vi "ChangeInheritanceDialog.vi"(0 "ClassWriterGOOP300 in":refnum<class "ClassWriterNative.lvclass">, 1 "LvClass":refnum<vi>, 5 "error in (no error)":errorcluster) -> (14 "ClassWriterGOOP300 out":refnum<class "ClassWriterNative.lvclass">, 15 "BaseClassPath":path, 16 "Cancelled":bool, 19 "error out":errorcluster)   [LabVIEW 2020, in "ClassWriterNative.lvclass"]
uses:
  ClassWriterNative.lvclass
  SubVIs/GOOP_HelpButton.ctl
panel:
  in  "Change inheritance to this class":string(combo)
  in  "_HelpChangeInheritance":T1
  in  "_Cancel":bool
  in  "_OK":bool
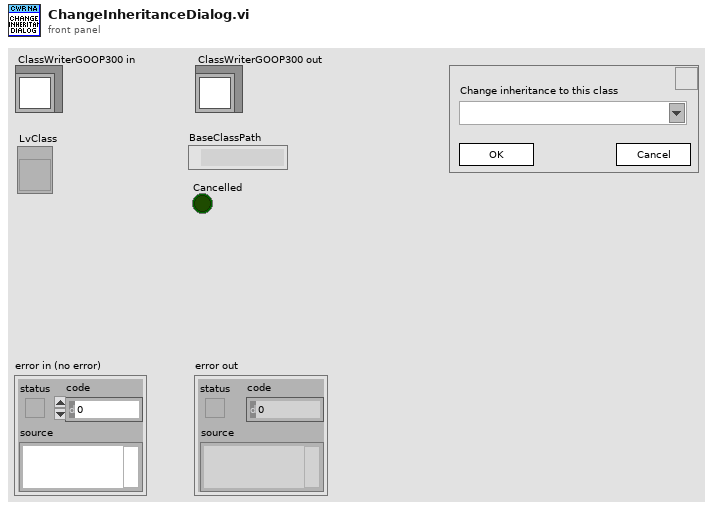
[diagram p1: front panel]
types:
  T1 = typedef "GOOP_HelpButton.ctl" = bool
  T2 = cluster{"LvClasses":refnum<vi>[], "ClassPathes":path[], "Cancelled":bool, "List":string[], "List index":i32}
  T3 = typedef "GDSLvCLass_ClassSettingsType.ctl" = cluster{"ClassProviderName":string, "ClassTemplateUsed":string, "ClassTemplateVersion":string, "ClassDescription":string, "PlugIns":T4[], "ConnectorPanePattern":string}
  T4 = typedef "GDSLvClass_PlugIn.ctl" = cluster{"Type":T5, "ID":string, "Version":string, "Path":path, "Name":string, "Data":variant}
  T5 = typedef "GDSLvClass_PlugInTypes.ctl" = enum16{"DesignPattern", "MethodTypes"}
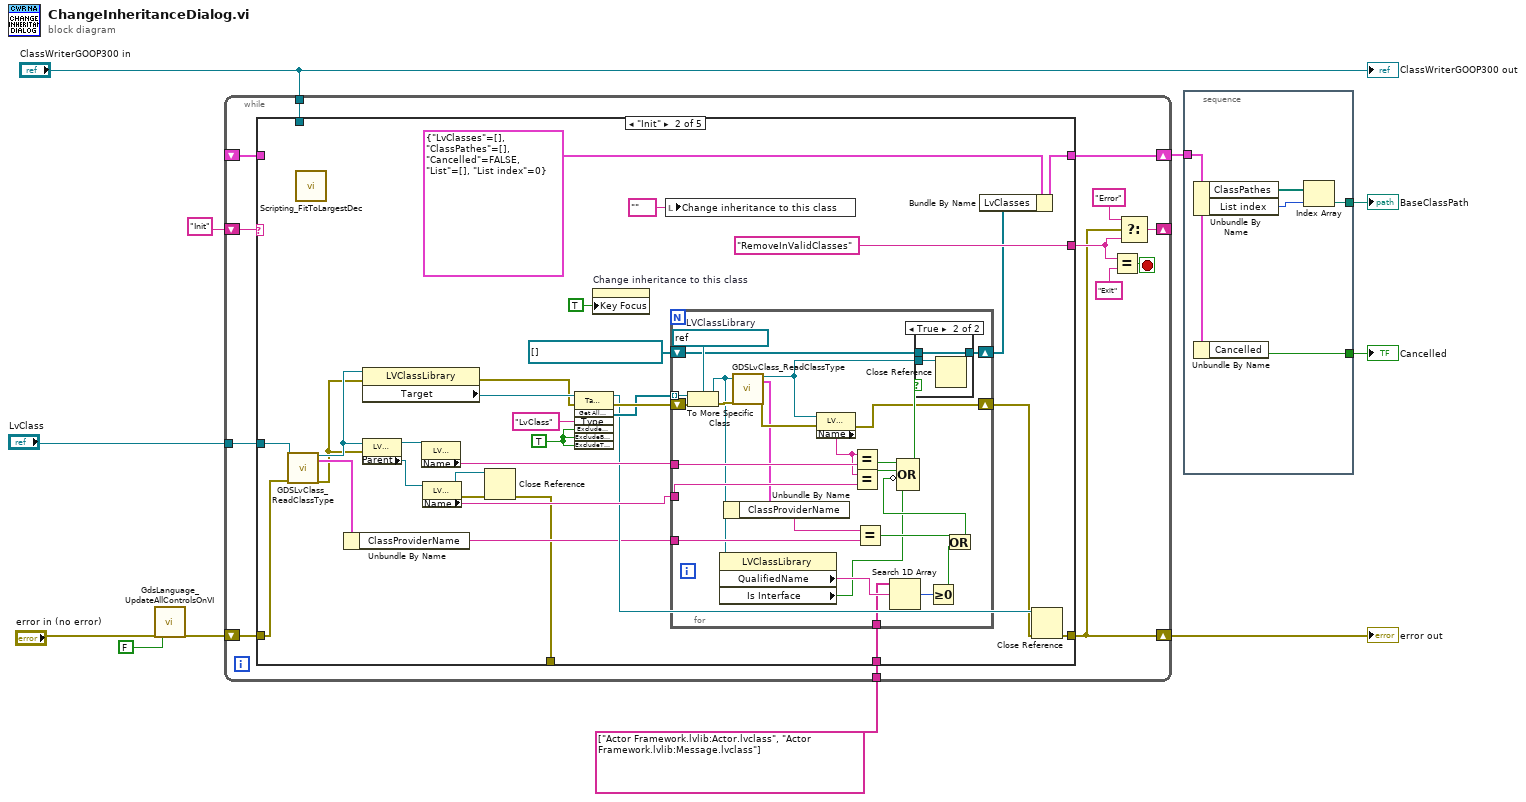
[diagram p0: block diagram]
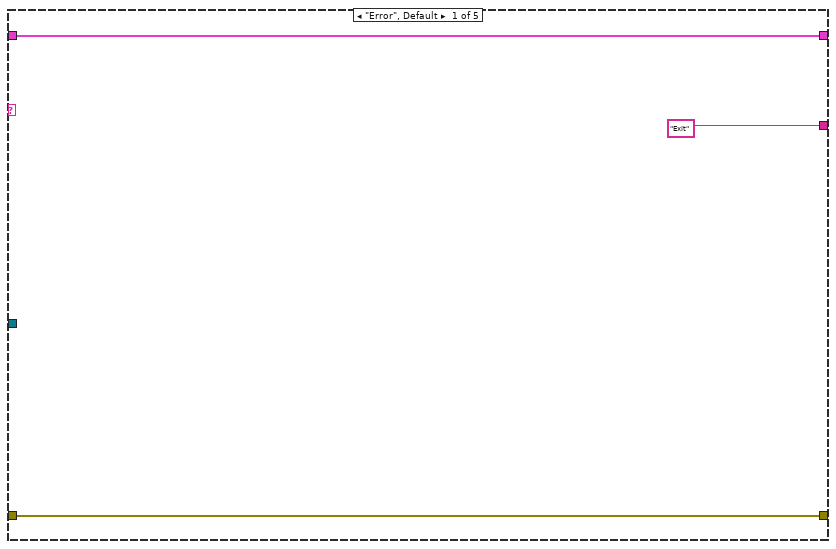
[diagram p2: hidden frame]
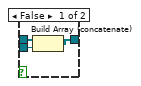
[diagram p3: hidden frame]
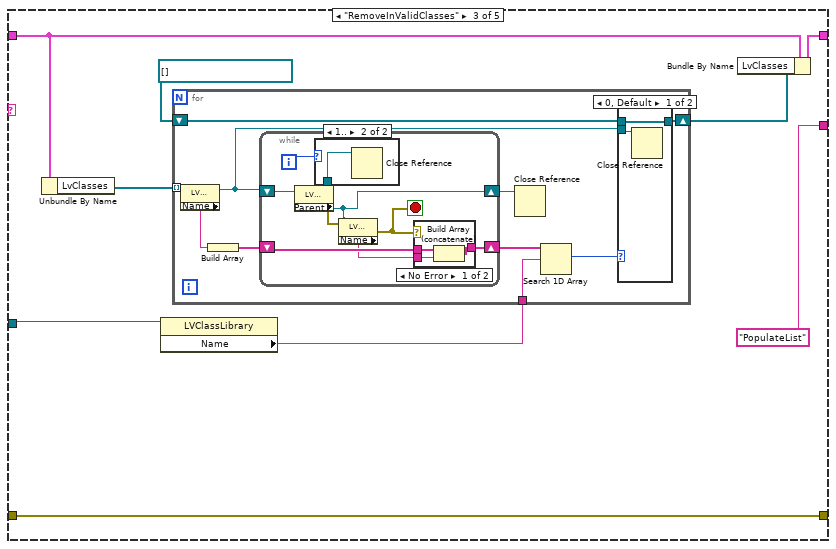
[diagram p4: hidden frame]
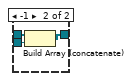
[diagram p5: hidden frame]
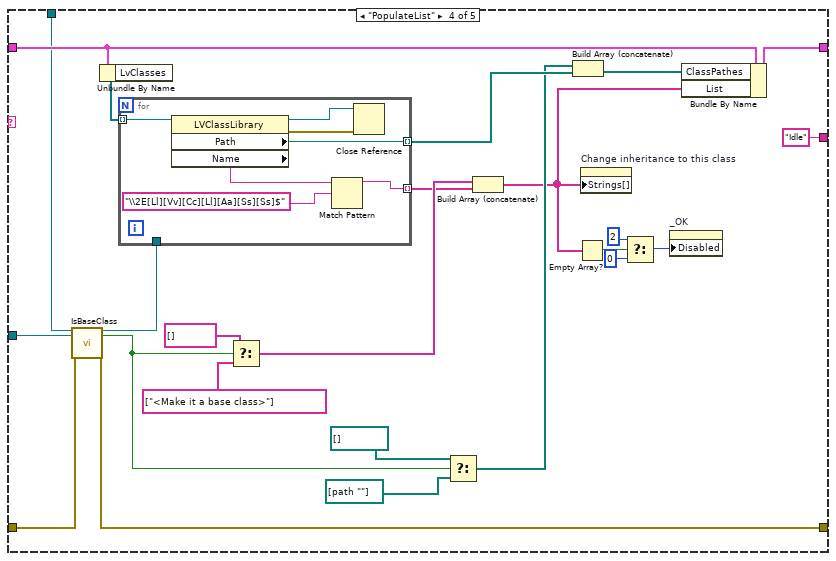
[diagram p8: hidden frame]
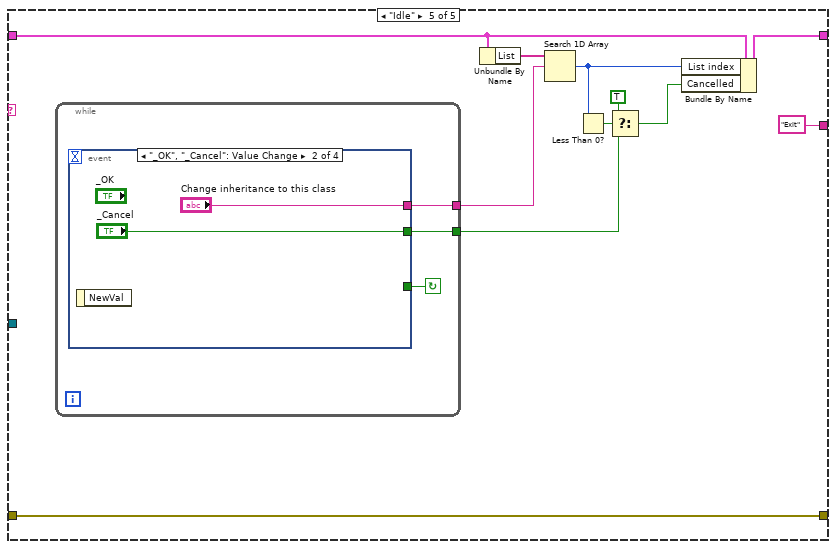
[diagram p9: hidden frame]
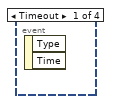
[diagram p10: hidden frame]
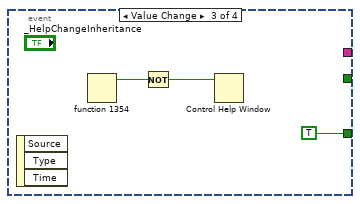
[diagram p11: hidden frame]
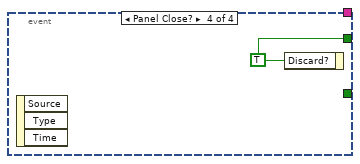
[diagram p12: hidden frame]
diagram:
  n1 = call "GdsLanguage_UpdateAllControlsOnVI.vi"("error in (no error)"="error in (no error)", "CreateLanguageFile(Use this to create a languageFile)"=FALSE) -> ("error out"=w6:errorcluster)  [unwired: 16 in, 1 out]
  n2 = while {
    shift-right: [w17] -> w2
    shift-left: w6 -> [w24]
    shift-right: [w22] -> _
    shift-left: "Init" -> [w23]
    shift-right: [w16] -> w9
    shift-left: _ -> [w15]
    tunnel: "LvClass" -> [w14]
    tunnel: "ClassWriterGOOP300 in" -> [w13]
    tunnel: string[] ["Actor Framework.lvlib:Actor.lvclass", "Actor Framework.lvlib:Message.lvclass"] -> [w12]
    stop <- w21 stop-if-true
    n3 = case shown="\"Init\"" w23 {
      tunnel: w24 -> [w27 w39 w89 w130 w168]
      tunnel: [w27 w42 w89 w129 w168] -> w17
      tunnel: ["Exit" "RemoveInValidClasses" "PopulateList" "Idle" "Exit"] -> w18
      tunnel: [w25 w50 w91 w143 w167] -> w16
      tunnel: w15 -> [w25 _ w93 w144 w165]
      tunnel: w14 -> [_ w40 w96 w132 _]
      tunnel: w13 -> [_ _ _ w131 _]
      tunnel: [_ w34 _ _ _] -> _
      tunnel: w12 -> [_ w30 _ _ _]
      frame "Error", Default {
      }
      frame "Init" {
        w49 = TRUE ("ExcludeDependencies")
        n4 = call "GDSLvClass_ReadClassType.vi"("Class Refnum In"=w40, "error in (no error)"=w39) -> ("Class Refnum Out"=w33:refnum<vi>, "ClassSettings"=w38:T3, "error out"=w32:errorcluster)  [unwired: 15 in]
        n5 = call "Scripting_FitToLargestDec.vi"() -> ()  [unwired: 6 in, 2 out]
        n6 = Unbundle By Name(w38) -> ("ClassProviderName"=w37:string)
        n7 = property class="LVClassLibrary"(reference=w33, error in=w32) -> (error out=w54:errorcluster, "Target"=w56:refnum<vi>)  [unwired: 1 out]
        n8 = property class="LVClassLibrary"(reference=w33, error in=w32) -> (reference out=w48:refnum<vi>, "Parent"=w47:refnum<vi>)  [unwired: 1 out]
        n9 = property class="LVClassLibrary"(reference=w48) -> ("Name"=w46:string)  [unwired: 1 in, 2 out]
        n10 = property class="LVClassLibrary"(reference=w47) -> (reference out=w35:refnum<vi>, error out=w36:errorcluster, "Name"=w45:string)  [unwired: 1 in]
        n11 = Close Reference(reference=w35, error in (no error)=w36) -> (error out=w34:errorcluster)
        n12 = invoke class="TargetItem" method="Get All Descendents"(reference=w56, error in=w54, "Type"="LvClass", "Exclude Dependencies"=w49, "ExcludeBuilds"=w49, "ExcludeTargets"=w49) -> (reference out=w41:refnum<vi>, error out=w53:errorcluster, "All Descendents"=w52:refnum<vi>[])  [unwired: 1 in, 4 out]
        n13 = property on="Change inheritance to this class" class="CmbBox"("Key Focus"=TRUE) -> ()  [unwired: 2 in, 2 out]
        n14 = local write "Change inheritance to this class"("" ("Change inheritance to this class")) -> ()
        n15 = for {
          shift-right: [w67] -> w31
          shift-left: w53 -> [w83]
          tunnel: w52 -> [w82] mode=indexing
          shift-right: [w73] -> w44
          shift-left: refnum<vi>[] [] -> [w74]
          tunnel: w46 -> [w80]
          tunnel: w45 -> [w78]
          tunnel: w37 -> [w68]
          tunnel: w30 -> [w63]
          w81 = refnum<vi> refnum  # LVClassLibrary
          n16 = To More Specific Class(target class=w81, reference=w82, error in=w83) -> (specific class reference=w65:refnum<vi>, error out=w70:errorcluster)
          n17 = property class="LVClassLibrary"(reference=w65) -> ("QualifiedName"=w64:string, "Is Interface"=w58:bool)  [unwired: 1 in, 2 out]
          n18 = call "GDSLvClass_ReadClassType.vi"("Class Refnum In"=w65, "error in (no error)"=w70) -> ("Class Refnum Out"=w71:refnum<vi>, "ClassSettings"=w66:T3, "error out"=w72:errorcluster)  [unwired: 15 in]
          n19 = Unbundle By Name(w66) -> ("ClassProviderName"=w69:string)
          n20 = property class="LVClassLibrary"(reference=w71, error in=w72) -> (error out=w67:errorcluster, "Name"=w79:string)  [unwired: 1 out]
          n21 = Equal?(x=w79, y=w80) -> (x = y?=w76:bool)
          n22 = Equal?(x=w79, y=w78) -> (x = y?=w77:bool)
          n23 = Equal?(x=w69, y=w68) -> (x = y?=w61:bool)
          n24 = Search 1D Array(1D array=w63, element=w64) -> (index of element=w62:i32)  [unwired: 1 in]
          n25 = Greater Or Equal To 0?(x=w62) -> (x >= 0?=w60:bool)
          n26 = Or(x=w61, y=w60) -> (x .or. y?=w59:bool)
          n27 = Compound Arithmetic op=OR(w76, w77, invert w59, w58) -> (w75:bool)
          n28 = case shown="True" w75 {
            tunnel: w74 -> [w86 w88]
            tunnel: [w85 w88] -> w73
            tunnel: w71 -> [w84 w87]
            frame False {
              n29 = Build Array (concatenate)(w86, w84) -> (w85:refnum<vi>[])
            }
            frame True {
              n30 = Close Reference(reference=w87) -> ()  [unwired: 1 in, 1 out]
            }
          }
        }
        n31 = Bundle By Name(cluster=T2 {"LvClasses"=[], "ClassPathes"=[], "Cancelled"=FALSE, "List"=[], "List index"=0}, "LvClasses"=w44) -> (w50:T2)
        n32 = Close Reference(reference=w41, error in (no error)=w31) -> (error out=w42:errorcluster)
      }
      frame "RemoveInValidClasses" {
        n33 = Unbundle By Name(w93) -> ("LvClasses"=w97:refnum<vi>[])
        n34 = property class="LVClassLibrary"(reference=w96) -> ("Name"=w95:string)  [unwired: 1 in, 2 out]
        n35 = for {
          tunnel: w97 -> [w107] mode=indexing
          tunnel: w95 -> [w102]
          shift-right: [w98] -> w92
          shift-left: refnum<vi>[] [] -> [w100]
          n36 = property class="LVClassLibrary"(reference=w107) -> (reference out=w99:refnum<vi>, "Name"=w105:string)  [unwired: 1 in, 1 out]
          n37 = Build Array(w105) -> (w104:string[])
          n38 = while {
            shift-right: [w115] -> w106
            shift-left: w99 -> [w121]
            shift-right: [w116] -> w103
            shift-left: w104 -> [w118]
            i -> [w113]
            stop <- w119 stop-if-true
            n39 = property class="LVClassLibrary"(reference=w121) -> (reference out=w114:refnum<vi>, error out=w120:errorcluster, "Parent"=w115:refnum<vi>)  [unwired: 1 in]
            n40 = case shown="1.." w113 {
              tunnel: w114 -> [_ w122]
              frame Default {
              }
              frame 1.. {
                n41 = Close Reference(reference=w122) -> ()  [unwired: 1 in, 1 out]
              }
            }
            n42 = property class="LVClassLibrary"(reference=w115, error in=w120) -> (error out=w119:errorcluster, "Name"=w117:string)  [unwired: 1 out]
            n43 = case shown="No Error" w119 {
              tunnel: w118 -> [w125 w126]
              tunnel: w117 -> [w124 _]
              tunnel: [w123 w126] -> w116
              frame No Error {
                n44 = Build Array (concatenate)(w125, w124) -> (w123:string[])
              }
              frame Error {
              }
            }
          }
          n45 = Close Reference(reference=w106) -> ()  [unwired: 1 in, 1 out]
          n46 = Search 1D Array(1D array=w103, element=w102) -> (index of element=w101:i32)  [unwired: 1 in]
          n47 = case shown="0, Default" w101 {
            tunnel: w100 -> [w108 w112]
            tunnel: w99 -> [w109 w111]
            tunnel: [w108 w110] -> w98
            frame 0, Default {
              n48 = Close Reference(reference=w109) -> ()  [unwired: 1 in, 1 out]
            }
            frame -1 {
              n49 = Build Array (concatenate)(w112, w111) -> (w110:refnum<vi>[])
            }
          }
        }
        n50 = Bundle By Name(cluster=w93, "LvClasses"=w92) -> (w91:T2)
      }
      frame "PopulateList" {
        n51 = call-dynamic "IsBaseClass.vi"("RefIn"=w131, "LvClass"=w132, "error in"=w130) -> ("RefOut"=w128:refnum<class "ClassWriterNative.lvclass">, "BaseClass"=w133:bool, "error out"=w129:errorcluster)  [unwired: 14 in]
        n52 = Unbundle By Name(w144) -> ("LvClasses"=w147:refnum<vi>[])
        n53 = for {
          tunnel: w147 -> [w157] mode=indexing
          tunnel: [w151] -> w146 mode=indexing
          tunnel: [w156] -> w142 mode=indexing
          tunnel: w128 -> [_]
          n54 = property class="LVClassLibrary"(reference=w157) -> (reference out=w154:refnum<vi>, error out=w155:errorcluster, "Path"=w156:path, "Name"=w153:string)  [unwired: 1 in]
          n55 = Match Pattern(string=w153, regular expression="\\2E[Ll][Vv][Cc][Ll][Aa][Ss][Ss]$") -> (before substring=w151:string)  [unwired: 1 in, 3 out]
          n56 = Close Reference(reference=w154, error in (no error)=w155) -> ()  [unwired: 1 out]
        }
        n57 = Select(t=string[] [], s=w133, f=string[] ["<Make it a base class>"] ("Strings []")) -> (s? t:f=w148:string[])
        n58 = Select(t=path[] [] ("array"), s=w133, f=path[] [path ""] ("array")) -> (s? t:f=w140:path[])
        n59 = Build Array (concatenate)(w148, w146) -> (w127:string[])
        n60 = Build Array (concatenate)(w140, w142) -> (w141:path[])
        n61 = Empty Array?(array=w127) -> (empty?=w137:bool)
        n62 = property on="Change inheritance to this class" class="CmbBox"("Strings[]"=w127) -> ()  [unwired: 2 in, 2 out]
        n63 = Select(t=u8 2 ("Disabled"), s=w137, f=u8 0) -> (s? t:f=w136:u8)
        n64 = property on="_OK" class="Bool"("Disabled"=w136) -> ()  [unwired: 2 in, 2 out]
        n65 = Bundle By Name(cluster=w144, "ClassPathes"=w141, "List"=w127) -> (w143:T2)
      }
      frame "Idle" {
        n66 = while {
          tunnel: [w171] -> w158
          tunnel: [w169] -> w163
          stop <- w170 continue-if-true
          n67 = event shown="[1] \"_OK\", \"_Cancel\": Value Change" {
            selector: _ -> [_ _ _ _]
            dyn-events: _ -> [_ _ _ _]
            timeout: _ -> [_ _ _ _]
            tunnel: [_ "_Cancel" _ w177] -> w171
            tunnel: [_ _ TRUE _] -> w170
            tunnel: [_ "Change inheritance to this class" _ _] -> w169
            event Timeout {
              n68 = event-data() -> ()  [unwired: 1 in, 2 out]
            }
            event "_OK", "_Cancel": Value Change {
              n69 = event-data() -> ()  [unwired: 1 in, 1 out]
            }
            event Value Change {
              n70 = event-data() -> ()  [unwired: 1 in, 3 out]
              n71 = fn#1354() -> (1:w175:bool)  [unwired: 1 out]
              n72 = Not(x=w175) -> (.not. x?=w174:bool)
              n73 = Control Help Window(1:w174) -> ()  [unwired: 1 in]
            }
            event Panel Close? {
              w177 = TRUE ("Discard?")
              n74 = event-data() -> ()  [unwired: 1 in, 3 out]
              n75 = event-data("Discard?"=w177) -> ()  [unwired: 1 in, 1 out]
            }
          }
        }
        n76 = Unbundle By Name(w165) -> ("List"=w164:string[])
        n77 = Search 1D Array(1D array=w164, element=w163) -> (index of element=w160:i32)  [unwired: 1 in]
        n78 = Less Than 0?(x=w160) -> (x < 0?=w161:bool)
        n79 = Select(t=TRUE, s=w161, f=w158) -> (s? t:f=w159:bool)
        n80 = Bundle By Name(cluster=w165, "List index"=w160, "Cancelled"=w159) -> (w167:T2)
      }
    }
    n81 = Equal?(x=w18, y="Exit") -> (x = y?=w21:bool)
    n82 = Select(t="Error", s=w17, f=w18) -> (s? t:f=w22:string)
  }
  "error out" <- w2
  n83 = stacked-sequence {
    tunnel: w9 -> [w182]
    tunnel: [w178] -> w8
    tunnel: [w180] -> w1
    frame #0 {
      n84 = Unbundle By Name(w182) -> ("ClassPathes"=w181:path[], "List index"=w179:i32)
      n85 = Unbundle By Name(w182) -> ("Cancelled"=w178:bool)
      n86 = Index Array(array=w181, index=w179) -> (element=w180:path)
    }
  }
  "Cancelled" <- w8
  "BaseClassPath" <- w1
  "ClassWriterGOOP300 out" <- "ClassWriterGOOP300 in"
